vi "UE_Stabilization_Reached.vi"(1 "threshold_ms":dbl, 2 "elapsed_ms":dbl) -> (0 "reached":bool)   [LabVIEW 2026]
doc: "INTENT: True when continuous-in-range duration equals or exceeds stabilization time. INPUTS: elapsed_ms (double), threshold_ms (double). OUTPUTS: reached (bool). DESIGN CONSTRAINT: This VI checks elapsed time. Reset and clock ownership belong to Step Tick. REQUIREMENTS: SRS-F-006. No physical hardware side effects. Acceptance requires native LabVIEW compilation and behavioral testing."
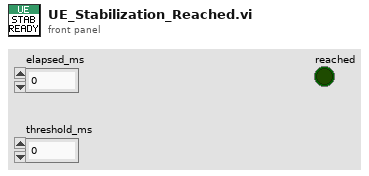
[diagram p1: front panel]
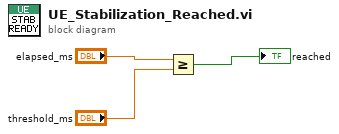
[diagram p0: block diagram]
diagram:
  n1 = Greater Or Equal?(x="elapsed_ms", y="threshold_ms") -> (x >= y?=→"reached":bool)
